vi "read_position_producerconsumer__31ba20afea.vi"(8 "error in (no error)":errorcluster, 10 "relative seconds":dbl, 11 "Refnum in":refnum<k21>) -> (0 "error out":errorcluster, 1 "time":dbl, 2 "data":dbl, 3 "Refnum out":refnum<k21>)   [LabVIEW 2023]
uses:
  <vilib>/DAQmx/read.llb/DAQmx Read (Analog DBL 1Chan 1Samp).vi
  <vilib>/DAQmx/miscellaneous.llb/DAQmx Fill In Error Info.vi
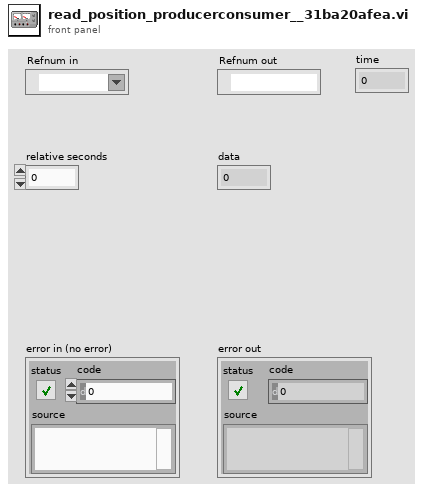
[diagram p1: front panel]
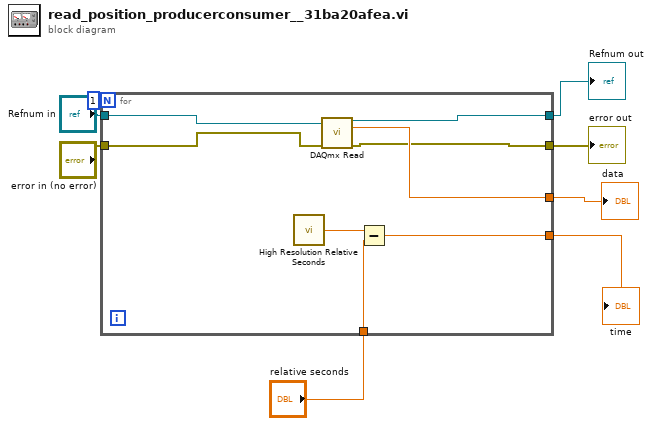
[diagram p0: block diagram]
diagram:
  n1 = for {
    N: 1 -> [_]
    tunnel: [w14] -> w3
    tunnel: "relative seconds" -> [w16]
    tunnel: "Refnum in" -> [w11]
    tunnel: [w12] -> w5
    tunnel: "error in (no error)" -> [w10]
    tunnel: [w13] -> w2
    tunnel: [w9] -> w1
    n2 = call <vilib>:"High Resolution Relative Seconds.vi"() -> ("relative seconds"=w15:dbl)
    n3 = call-poly <vilib>:"DAQmx Read.vi"("task/channels in"=w11, "error in"=w10) -> ("task out"=w12:refnum<k21>, "data"=w14:dbl, "error out"=w13:errorcluster)  [unwired: 11 in]
    n4 = Subtract(x=w15, y=w16) -> (x-y=w9:dbl)
  }
  "Refnum out" <- w5
  "data" <- w3
  "error out" <- w2
  "time" <- w1
